vi "lvmcp_bounds.vi"() -> ()   [LabVIEW 2026]
panel:
  out "error out":errorcluster
  out "bounds":cluster{"Area Width":i32, "Area Height":i32}
  out "position":cluster{"Left":i32, "Top":i32}
  in  "reference":refnum<vi>
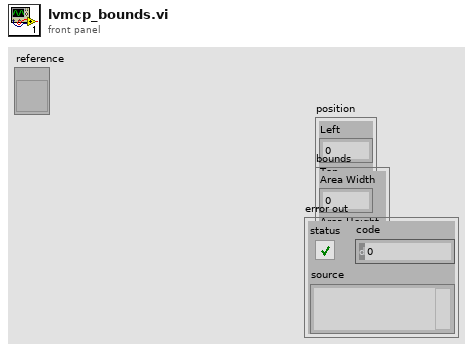
[diagram p1: front panel]
types:
  T1 = typedef "LVPositionTypeDef.ctl" = cluster{"Left":i32, "Top":i32}
  T2 = typedef "LVBoundsTypeDef.ctl" = cluster{"Width":u32, "Height":u32}
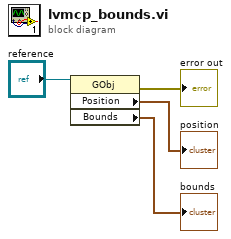
[diagram p0: block diagram]
diagram:
  n1 = property class="GObj"(reference="reference") -> (error out=→"error out":errorcluster, "Position"=→"position":T1, "Bounds"=→"bounds":T2)  [unwired: 1 in, 1 out]
